vi "FPGA Video Recording (Host).vi"() -> ()   [LabVIEW 2013]
doc: "This is the host VI for the 10-Tap 8-Bit Camera with DRAM example. This example demonstrates how to acquire images from a 10-tap, 8-bit, extended configuration, Camera Link camera and display the images on the host. This example supports area scan and line scan cameras for both continuous and finite acquisitions.\n\nThis example also demonstrates the use of DRAM as a frame buffer for very high speed acquisitions. Data packing and flow-control are also employed to maximize use of the available DRAM and FIFOs in terms of both memory space and performance.\n\nAdditionally, the example demonstrates the serial server, which allows third-party camera configuration utilities to communicate with the camera using the Camera Link serial interface while this VI is running."
uses:
  <vilib>/userdefined/High Color/nirio_resource_hc.ctl
  <vilib>/vision/Avi.llb/IMAQ AVI2 Refnum.ctl
  <vilib>/rvi/interface/common/niFpgaWaitOnOcc.vi
  <vilib>/FPGAPlugInAG/PCIe-1473R-LX110/niLvFpga_Open_PCIe-1473R-LX110.vi
  <vilib>/rvi/interface/common/dynamic/niFpgaDynamicAddResources.vi
  <vilib>/FPGAPlugInAG/Dynamic/niLvFpga_Reset_Dynamic.vi
  <vilib>/Utility/error.llb/Error Cluster From Error Code.vi
  <vilib>/rvi/errors/niLvFpgaAdjustHostInterfaceError.vi
  <vilib>/FPGAPlugInAG/Dynamic/niLvFpga_Run_Dynamic.vi
  <vilib>/FPGAPlugInAG/Dynamic/niLvFpga_Close_Dynamic.vi
  <vilib>/rvi/interface/nirviOpenFPGA/nirviOpenFPGA.xnode
  Vision-RIO/10-Tap 8-bit Camera with DRAM/FPGA Bitfiles/10-Tap8-bitCameraWithDRAMModifiedLX110.lvbitx
  <vilib>/rvi/interface/nirviMethod/nirviMethod.xnode
  <vilib>/rvi/interface/nirviReadWriteControl/nirviReadWriteControl.xnode
  <vilib>/rvi/interface/nirviCloseFPGA/nirviCloseFPGA.xnode
  <vilib>/rvi/interface/Simulation/niFpgaSimulationCallBeginRW.vi
  <vilib>/rvi/errors/niLvFpgaMergeErrorWithErrorCode.vi
  NiFpgaLv.dll
  <vilib>/FPGAPlugInAG/Dynamic/niLvFpga_ConfigureFifo_Dynamic.vi
  <vilib>/FPGAPlugInAG/Dynamic/niLvFpga_StartFifo_Dynamic.vi
  <vilib>/FPGAPlugInAG/Dynamic/niLvFpga_ReadFifo_Dynamic.vi
panel:
  out "Elements Remaining":u32
  out "DMA Full":bool
  out "Codec Chosen":string="Motion JPEG (NI Vision)"
  in  "Codec index":i32=4
  out "Installed Codecs":string[](array[string])=["Microsoft Video 1", "Intel IYUV codec", "Cinepak Codec by Radius", "FF Video Codec 1 (FFV1) (NI Vision)", "Motion JPEG (NI Vision)", "Y800 Uncompressed Grey Scale (NI Vision)", "YUV 4:2:0 Planar (NI Vision)"]
  out "AVI Path":path=path "F:/Live_Data/201310230_saveFPGAframes/test10.avi"
  in  "AVI fps":u32=200
  out "# of lost frames":u32
  in  "Record?":bool=TRUE
  in  "DMA Buffer Size\n(In Images)":u32=2200 caption="DMA Buffer Size \n       (Frames)"
  in  "Signal Mapping":T1(ring)=enum."Basler 10-tap"
  out "Acq In Progress":bool
  in  "Line Scan":bool
  in  "Frames To Acquire":u32=2000 caption="Frames To Acquire\n(0 = infinite)"
  in  "Cancel":bool
  out "Acq'd Frame Width":u32=1200
  in  "Stopped":bool=TRUE
  in  "RIO Device":T2="RIO0"
  out "DMA Write Timeout":bool
  in  "Start Serial Server":bool=TRUE
  out "Frames Acq'd":u32=2000
  out "Acq'd Frame Height":u32=788
  out "Image":T3(plugin-control)
  in  "Acquire":bool
  in  "Stop":bool
  in  "Image Height":u32=788 max=65535
  in  "Image Width":u32=1200 max=65535 step=40
  out "Initialized":bool
  # "Set the Camera to 10-Tap and AOI to 1200 x 788"
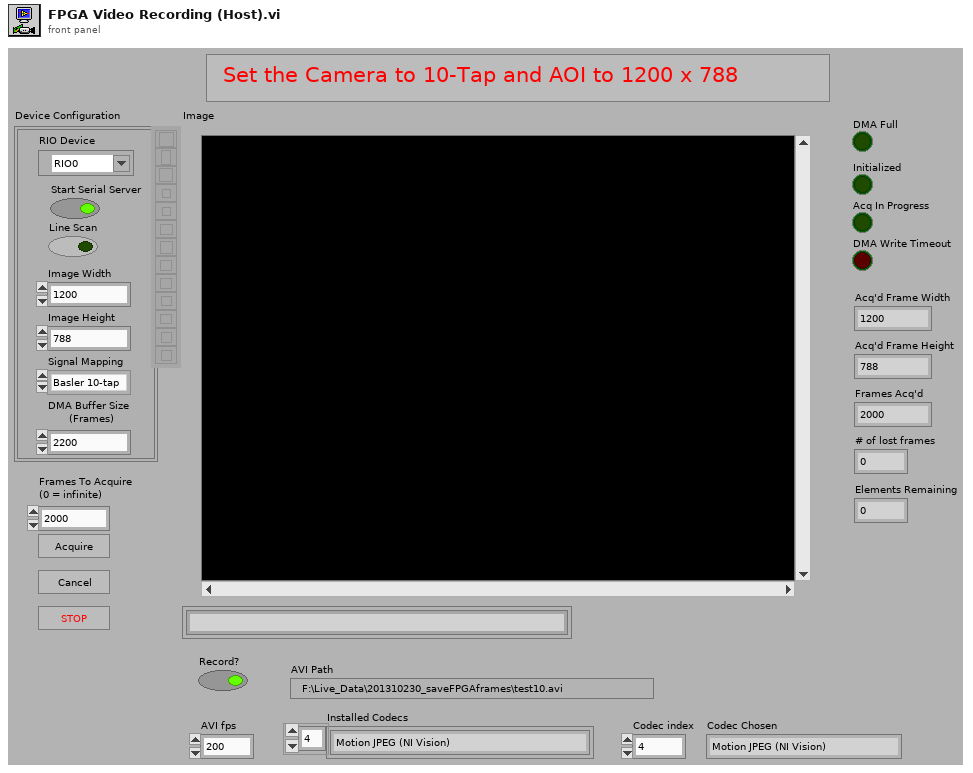
[diagram p1: front panel]
types:
  T1 = enum8{"Standard", "Basler 10-tap", "Vosskühler 10-tap"}
  T2 = typedef "nirio_resource_hc.ctl" = tag
  T3 = typedef "IMAQ Image.ctl" = refnum<image>
  T4 = typedef "Image Type" = u32
  T5 = typedef "IMAQ AVI2 Refnum.ctl" = refnum<k20>
  T6 = enum16{"big-endian, network order", "native, host order", "little-endian"}
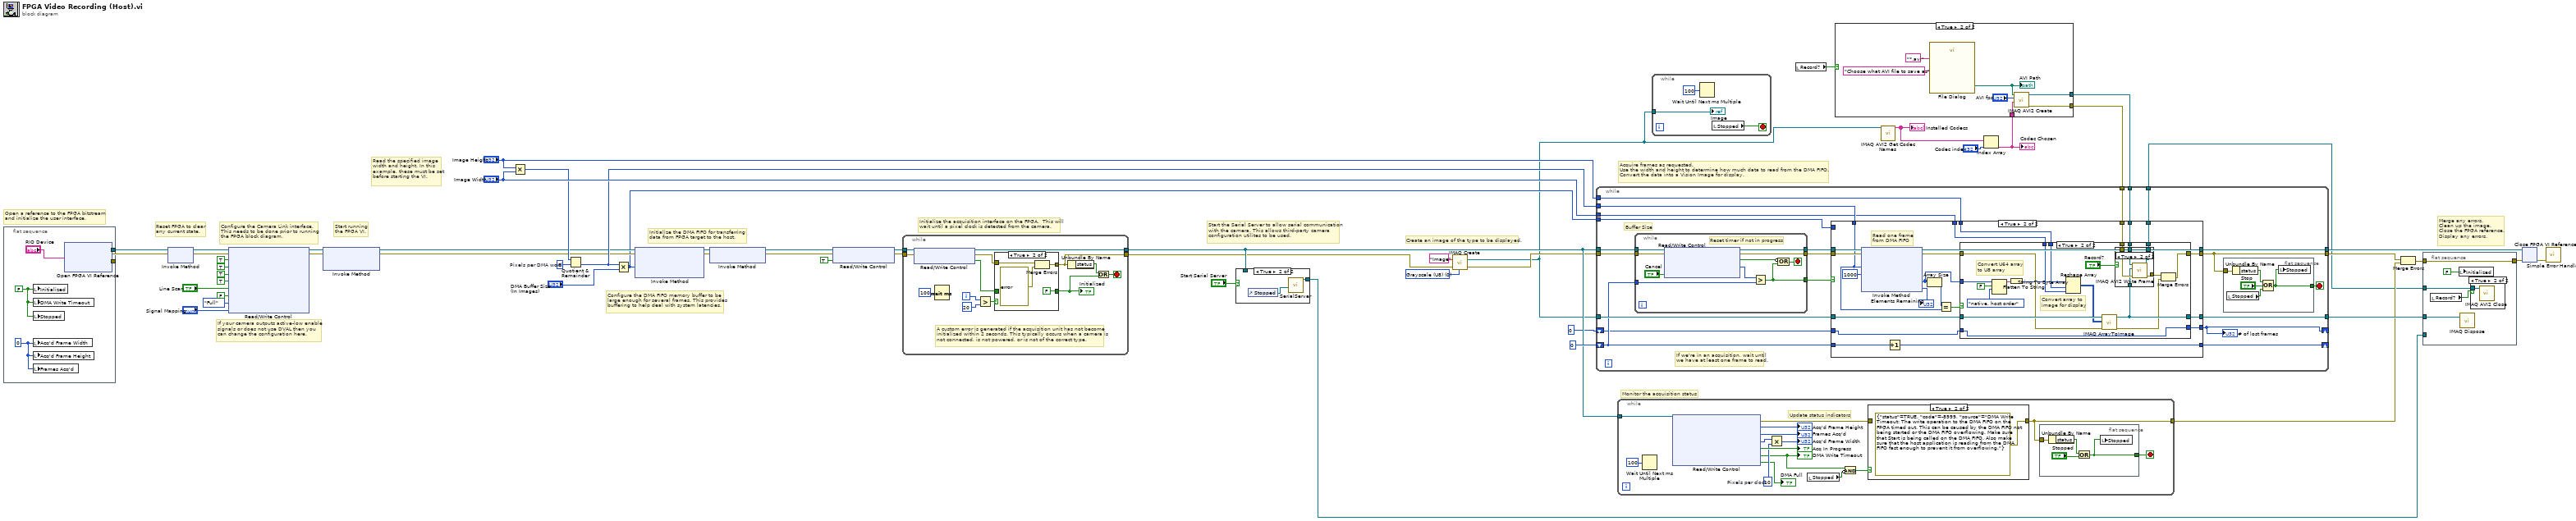
[diagram p0: block diagram]
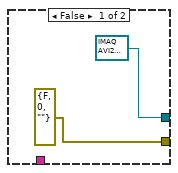
[diagram p2: hidden frame]
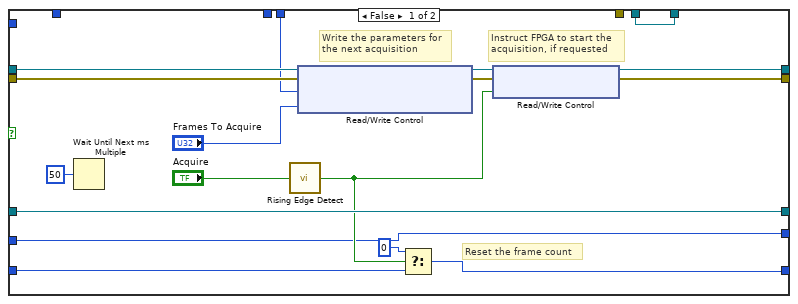
[diagram p6: hidden frame]
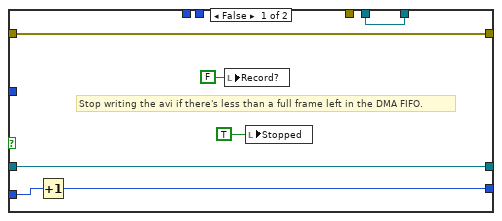
[diagram p7: hidden frame]
diagram:
  w16 = u32 8  # Pixels per DMA word
  w50 = T4 0 items=["Grayscale (U8)", "Grayscale (I16)", "Grayscale (SGL)", "Complex (CSG)", "RGB (U32)", "HSL (U32)", "RGB (U64)", "Grayscale (U16)"] ("Image Type")
  # "If your camera outputs active-low enable\nsignals or does not use DVAL then you \ncan change the configuration here."
  # "Configure the DMA FIFO memory buffer to be\nlarge enough for several frames. This provides\nbuffering to help deal with system latencies."
  # "Start running\nthe FPGA VI."
  # "Reset FPGA to clear\nany current state."
  # "Read the specified image\nwidth and height. In this\nexample, these must be set\nbefore starting the VI."
  # "Merge any errors.\nClean up the image.\nClose the FPGA reference.\nDisplay any errors."
  # "Acquire frames as requested.\nUse the width and height to determine how much data to read from the DMA FIFO.\nConvert the data into a Vision Image for display."
  # "Monitor the acquisition status"
  # "Start the Serial Server to allow serial communication\nwith the camera. This allows third-party camera\nconfiguration utilites to be used."
  # "Create an image of the type to be displayed."
  # "Initialize the acquisition interface on the FPGA.  This will\nwait until a pixel clock is detected from the camera."
  # "Initialize the DMA FIFO for transferring\ndata from FPGA target to the host."
  # "Configure the Camera Link interface.\nThis needs to be done prior to running\nthe FPGA block diagram."
  # "Open a reference to the FPGA bitstream\nand initialize the user interface."
  n1 = flat-sequence {
    tunnel: [w57] -> w41
    tunnel: [w56] -> w54
    frame #0 {
      w59 = u32 0 ("Num Lines Acq'd")
      w58 = FALSE ("stop")
      n2 = local write "Initialized"(w58) -> ()
      n3 = local write "DMA Write Timeout"(w58) -> ()
      n4 = local write "Stopped"(w58) -> ()
      n5 = local write "Acq'd Frame Width"(w59) -> ()
      n6 = local write "Acq'd Frame Height"(w59) -> ()
      n7 = local write "Frames Acq'd"(w59) -> ()
      n8 = xnode "Open FPGA VI Reference"("resource name"="RIO Device") -> ("FPGA VI Reference Out"=w57:refnum<k20>, "error out"=w56:errorcluster)  [unwired: 1 in]
    }
  }
  n9 = xnode "Invoke Method"("FPGA VI Reference In"=w41, "error in"=w54) -> ("FPGA VI Reference Out"=w30:refnum<k20>, "error out"=w33:errorcluster)
  n10 = xnode "Read/Write Control"("FPGA VI Reference In"=w30, "error in"=w33, "CL Config.FVAL Active High"=TRUE ("IO Module Config.CL FVAL Active High"), "CL Config.LVAL Active High"=TRUE ("IO Module Config.CL LVAL Active High"), "CL Config.DVAL Active High"=TRUE ("IO Module Config.CL DVAL Active High"), "CL Config.Spare Active High"=TRUE ("IO Module Config.CL Spare Active High"), "CL Config.Line Scan"="Line Scan", "Acq Control.Ignore DVAL"=FALSE ("CL Config.Line Scan"), "CL Config.Configuration"=enum8{"Base", "Medium", "Full"}."Full", "CL Config.Signal Mapping"="Signal Mapping") -> ("FPGA VI Reference Out"=w34:refnum<k20>, "error out"=w32:errorcluster)
  n11 = xnode "Invoke Method"("FPGA VI Reference In"=w34, "error in"=w32) -> ("FPGA VI Reference Out"=w13:refnum<k20>, "error out"=w12:errorcluster)  [unwired: 1 in]
  n12 = Multiply(x="Image Height", y="Image Width") -> (x*y=w15:u32)
  n13 = Quotient & Remainder(x=w15, y=w16) -> (floor(x/y)=w14:u32)  [unwired: 1 out]
  n14 = Multiply(x=w14, y="DMA Buffer Size\n(In Images)") -> (x*y=w9:u32)
  n15 = xnode "Invoke Method"("FPGA VI Reference In"=w13, "error in"=w12, "Requested Depth"=w9) -> ("FPGA VI Reference Out"=w40:refnum<k20>, "error out"=w39:errorcluster)  [unwired: 1 out]
  n16 = xnode "Invoke Method"("FPGA VI Reference In"=w40, "error in"=w39) -> ("FPGA VI Reference Out"=w25:refnum<k20>, "error out"=w38:errorcluster)
  n17 = xnode "Read/Write Control"("FPGA VI Reference In"=w25, "error in"=w38, "Acq Control.Initialize"=TRUE ("Arm Acquisition")) -> ("FPGA VI Reference Out"=w53:refnum<k20>, "error out"=w52:errorcluster)
  n18 = while {
    tunnel: w53 -> [w67]
    tunnel: w52 -> [w66]
    tunnel: [w65] -> w22
    tunnel: [w69] -> w21
    i -> [w61]
    stop <- w72 stop-if-true
    # "A custom error is generated if the acquisition unit has not become\ninitialized within 2 seconds. This typically occurs when a camera is\nnot connected, is not powered, or is not of the correct type."
    n19 = xnode "Read/Write Control"("FPGA VI Reference In"=w67, "error in"=w66) -> ("FPGA VI Reference Out"=w65:refnum<k20>, "error out"=w64:errorcluster, "Acq Status.Initialized"=w63:bool)
    n20 = Wait (ms)(milliseconds to wait=u32 100) -> ()  [unwired: 1 out]
    n21 = Greater?(x=w61, y=20) -> (0:w62:bool)
    n22 = case shown="True" w62 {
      tunnel: [w74 FALSE] -> w68
      tunnel: w63 -> [w74 _]
      tunnel: w64 -> [w73 w76]
      tunnel: [w73 w78] -> w69
      frame False {
      }
      frame True {
        n23 = Merge Errors(w76, errorcluster {"status"=TRUE, "code"=-8999, "source"="Acquisition Initialization: This error typically occurs when a camera is not properly connected, is not powered, or is not of the correct type."} ("error in")) -> (w78:errorcluster)
      }
    }
    "Initialized" <- w68
    n24 = Unbundle By Name(w69) -> ("status"=w71:bool)
    n25 = Or(x=w71, y=w68) -> (x .or. y?=w72:bool)
  }
  n26 = case shown="True" "Start Serial Server" {
    tunnel: [_ w79] -> w42
    tunnel: w22 -> [_ _]
    frame False {
    }
    frame True {
      n27 = control-ref of="Stopped"() -> (w80:refnum<vi>)
      n28 = call "SerialServer.vi"("Stop Refnum"=w80) -> ("FPGA VI Reference Out"=w79:refnum<k20>)  [unwired: 6 in]
    }
  }
  n29 = call "IMAQ Create"("Image Name"="Image", "Image Type"=w50, "error in (no error)"=w21) -> ("New Image"=w5:T3, "error out"=w11:errorcluster)  [unwired: 2 in]
  n30 = while {
    tunnel: w22 -> [w92]
    tunnel: [w95] -> w35
    stop <- w94 stop-if-true
    w85 = u32 10  # Pixels per clock
    # "Update status indicators"
    n31 = Wait Until Next ms Multiple(millisecond multiple=u32 100) -> ()  [unwired: 1 out]
    n32 = xnode "Read/Write Control"("FPGA VI Reference In"=w92) -> ("error out"=w91:errorcluster, "Acq Status.Lines Per Frame"=→"Acq'd Frame Height":u32, "Acq Status.Frames Acq'd"=→"Frames Acq'd":u32, "Acq Status.Clocks Per Line"=w86:u32, "Acq Status.Acq In Progress"=→"Acq In Progress":bool, "Acq Status.DMA Write Timeout"=w83:bool, "DMA Full?"=→"DMA Full":bool)  [unwired: 1 in, 1 out]
    "DMA Write Timeout" <- w83
    n33 = Multiply(x=w86, y=w85) -> (x*y=→"Acq'd Frame Width":u32)
    n34 = local read "Stopped"() -> (w82:bool)
    n35 = Compound Arithmetic op=AND(w83, invert w82) -> (w84:bool)
    n36 = case shown="True" w84 {
      tunnel: w91 -> [w100 _]
      tunnel: [w100 errorcluster {"status"=TRUE, "code"=-8999, "source"="DMA Write Timeout: The write operation to the DMA FIFO on the FPGA timed out. This can be caused by the DMA FIFO not being started or the DMA FIFO overflowing. Make sure that Start is being called on the DMA FIFO. Also make sure that the host application is reading from the DMA FIFO fast enough to prevent it from overflowing."} ("error out")] -> w95
      frame False {
      }
      frame True {
      }
    }
    n37 = flat-sequence {
      tunnel: w95 -> [w99]
      tunnel: [w97] -> w94
      frame #0 {
        n38 = Unbundle By Name(w99) -> ("status"=w98:bool)
        n39 = Or(x=w98, y="Stopped") -> (x .or. y?=w97:bool)
        n40 = local write "Stopped"(w97) -> ()
      }
    }
  }
  n41 = while {
    tunnel: w5 -> [w104]
    stop <- w102 stop-if-true
    n42 = Wait Until Next ms Multiple(millisecond multiple=u32 100) -> ()  [unwired: 1 out]
    n43 = local read "Stopped"() -> (w102:bool)
    "Image" <- w104
  }
  n44 = local read "Record?"() -> (w1:bool)
  n45 = call "IMAQ AVI2 Get Codec Names"("Image"=w5) -> ("Codec Names"=w6:string[])  [unwired: 9 in, 1 out]
  "Installed Codecs" <- w6
  n46 = Index Array(array=w6, index="Codec index") -> (element=w7:string)
  "Codec Chosen" <- w7
  n47 = case shown="True" w1 {
    tunnel: w7 -> [_ w113]
    tunnel: [T5 refnum ("AVI Refnum") w108] -> w4
    tunnel: [errorcluster {"status"=FALSE, "code"=0, "source"=""} ("error out") w107] -> w3
    frame False {
    }
    frame True {
      n48 = call "File Dialog"("prompt"="Choose what AVI file to save as", "pattern (all files)"="*.avi" ("pattern label")) -> ("selected path"=w112:path)  [unwired: 10 in, 3 out]
      "AVI Path" <- w112
      n49 = call "IMAQ AVI2 Create"("Codec"=w113, "Frames Per Second"="AVI fps", "AVI Path"=w112) -> ("error out"=w107:errorcluster, "AVI Refnum"=w108:T5)  [unwired: 7 in]
    }
  }
  n50 = while {
    tunnel: w22 -> [w126]
    tunnel: w11 -> [w125]
    tunnel: w14 -> [w134]
    tunnel: "Image Height" -> [w133]
    tunnel: "Image Width" -> [w132]
    tunnel: w5 -> [w131]
    tunnel: [w129] -> w36
    tunnel: [w130] -> w49
    tunnel: [w127] -> w44
    shift-right: [w121] -> _
    shift-left: u32 0 -> [w120]
    shift-right: [w119] -> _
    shift-left: u32 0 -> [w118]
    tunnel: w9 -> [w117]
    tunnel: w4 -> [w116]
    tunnel: w3 -> [w115]
    tunnel: [w114] -> w2
    stop <- w128 stop-if-true
    # "Buffer Size"
    # "If we're in an acquisition, wait until\nwe have at least one frame to read."
    n51 = while {
      tunnel: w126 -> [w141]
      tunnel: w125 -> [w140]
      tunnel: [w138] -> w124
      tunnel: [w139] -> w123
      tunnel: w120 -> [w144]
      tunnel: [w142] -> w122
      stop <- w143 stop-if-true
      # "Reset timer if not in progress"
      n52 = xnode "Read/Write Control"("FPGA VI Reference In"=w141, "error in"=w140, "Acq Control.Cancel Acq"="Cancel") -> ("FPGA VI Reference Out"=w139:refnum<k20>, "error out"=w138:errorcluster, "Acq Status.Acq In Progress"=w135:bool, "Acq Status.Frames Acq'd"=w137:u32)
      n53 = Greater?(x=w137, y=w144) -> (0:w142:bool)
      n54 = Compound Arithmetic op=OR(invert w135, w142) -> (w143:bool)
    }
    n55 = case shown="True" w122 {
      tunnel: w123 -> [w162 w181]
      tunnel: w124 -> [w161 w180]
      tunnel: w134 -> [_ w170]
      tunnel: w133 -> [w155 w188]
      tunnel: w132 -> [_ w187]
      tunnel: w131 -> [w166 w186]
      tunnel: [w157 w184] -> w129
      tunnel: [w160 w183] -> w130
      tunnel: [w166 w182] -> w127
      tunnel: w120 -> [w163 w179]
      tunnel: [w165 w178] -> w121
      tunnel: [w151 w177] -> w119
      tunnel: w118 -> [w151 w176]
      tunnel: w117 -> [_ _]
      tunnel: w116 -> [w150 w175]
      tunnel: w115 -> [_ w174]
      tunnel: [w150 w173] -> w114
      frame False {
        # "Reset the frame count"
        # "Instruct FPGA to start the\nacquisition, if requested"
        # "Write the parameters for\nthe next acquisition"
        n56 = Wait Until Next ms Multiple(millisecond multiple=u32 50) -> ()  [unwired: 1 out]
        n57 = call "Rising Edge Detect.vi"("Input"="Acquire") -> ("Pulse"=w152:bool)  [unwired: 4 in]
        n58 = xnode "Read/Write Control"("FPGA VI Reference In"=w162, "error in"=w161, "Acq Control.Line Scan Height"=w155, "Acq Control.Frames To Acq"="Frames To Acquire") -> ("FPGA VI Reference Out"=w159:refnum<k20>, "error out"=w158:errorcluster)
        n59 = Select(t=u32 0, s=w152, f=w163) -> (s? t:f=w165:u32)
        n60 = xnode "Read/Write Control"("FPGA VI Reference In"=w159, "error in"=w158, "Acq Control.Acquire"=w152) -> ("FPGA VI Reference Out"=w160:refnum<k20>, "error out"=w157:errorcluster)
      }
      frame True {
        # "Read one frame\nfrom DMA FIFO"
        n61 = xnode "Invoke Method"("FPGA VI Reference In"=w181, "error in"=w180, "Number of Elements"=w170, "Timeout (ms)"=1000) -> ("FPGA VI Reference Out"=w183:refnum<k20>, "error out"=w185:errorcluster, "Data"=w168:u64[], "Elements Remaining"=→"Elements Remaining":u32)
        n62 = Increment(x=w179) -> (x+1=w178:u32)
        n63 = Array Size(array=w168) -> (size(s)=w171:i32)
        n64 = Equal?(x=w171, y=w170) -> (x = y?=w169:bool)
        n65 = case shown="True" w169 {
          tunnel: w188 -> [_ w214]
          tunnel: w187 -> [_ w213]
          tunnel: w186 -> [w195 w212]
          tunnel: w185 -> [w194 w211]
          tunnel: [w194 w197] -> w184
          tunnel: [w195 w204] -> w182
          tunnel: w168 -> [_ w208]
          tunnel: [w193 w202] -> w177
          tunnel: w176 -> [w192 w202]
          tunnel: w175 -> [w190 w201]
          tunnel: w174 -> [_ w200]
          tunnel: [w190 w196] -> w173
          frame False {
            # "Stop writing the avi if there's less than a full frame left in the DMA FIFO."
            n66 = Increment(x=w192) -> (x+1=w193:u32)
            n67 = local write "Record?"(FALSE ("Record?")) -> ()
            n68 = local write "Stopped"(TRUE ("Stop")) -> ()
          }
          frame True {
            # "Convert U64 array\nto U8 array"
            # "Convert array to\nimage for display"
            n69 = Flatten To String(anything=w208, prepend array or string size? (T)=FALSE, byte order (0:big-endian, network order)=T6."native, host order") -> (data string=w206:string)  [unwired: 1 in, 2 out]
            n70 = String To Byte Array(string=w206) -> (unsigned byte array=w205:u8[])
            n71 = Reshape Array(w205, w214, w213) -> (w210:u8[][])
            n72 = call "IMAQ ArrayToImage"("error in (no error)"=w211, "Image Pixels (U8)"=w210, "Image"=w212) -> ("error out"=w198:errorcluster, "Image Out"=w204:T3)  [unwired: 7 in]
            n73 = case shown="True" "Record?" {
              tunnel: w204 -> [_ w219]
              tunnel: [w216 w218] -> w199
              tunnel: w201 -> [w215 w221]
              tunnel: w200 -> [w216 w220]
              tunnel: [w215 w217] -> w196
              frame False {
              }
              frame True {
                n74 = call "IMAQ AVI2 Write Frame"("error in (no error)"=w220, "Image"=w219, "AVI Refnum"=w221) -> ("error out"=w218:errorcluster, "AVI Refnum (duplicate)"=w217:T5)  [unwired: 6 in, 1 out]
              }
            }
            n75 = Merge Errors(w199, w198) -> (w197:errorcluster)
          }
        }
      }
    }
    "# of lost frames" <- w119
    n76 = flat-sequence {
      tunnel: w129 -> [w147]
      tunnel: [w146] -> w128
      frame #0 {
        n77 = local read "Stopped"() -> (w145:bool)
        n78 = Unbundle By Name(w147) -> ("status"=w148:bool)
        n79 = Compound Arithmetic op=OR(w148, "Stop", w145) -> (w146:bool)
        n80 = local write "Stopped"(w146) -> ()
      }
    }
  }
  n81 = Merge Errors(w36, w35) -> (w37:errorcluster)
  n82 = flat-sequence {
    tunnel: w37 -> [w225]
    tunnel: [w225] -> w46
    tunnel: w44 -> [w226]
    tunnel: w42 -> [_]
    tunnel: w2 -> [w223]
    frame #0 {
      n83 = local read "Record?"() -> (w222:bool)
      n84 = local write "Initialized"(FALSE ("Module Enabled")) -> ()
      n85 = call "IMAQ Dispose"("Image"=w226) -> ()  [unwired: 5 in, 1 out]
      n86 = case shown="True" w222 {
        tunnel: w223 -> [_ w227]
        frame False {
        }
        frame True {
          n87 = call "IMAQ AVI2 Close"("AVI Refnum"=w227) -> ()  [unwired: 10 in, 1 out]
        }
      }
    }
  }
  n88 = xnode "Close FPGA VI Reference"("FPGA VI Reference In"=w49, "error in"=w46) -> ("error out"=w43:errorcluster)
  n89 = call <vilib>:"Simple Error Handler.vi"("error in (no error)"=w43) -> ()  [unwired: 4 in, 5 out]
